vi "Export.vi"(8 "error in (no error)":errorcluster, 11 "Test Report.Template in":refnum<class "Test Report.Template.lvclass">) -> (0 "error out":errorcluster, 3 "Test Report.Template out":refnum<class "Test Report.Template.lvclass">)   [LabVIEW 2020, in "Caraya.lvlib" / "Test Report.Template.lvclass"]
uses:
  Test Report.Template.lvclass
  C:/projects/caraya/src/classes/Test Report/Test Report.lvclass
  Test Report.Template.lvclass/Test Report.Template.ctl
  Test Report/Test Report.lvclass
  Test Result/Test Result.lvclass
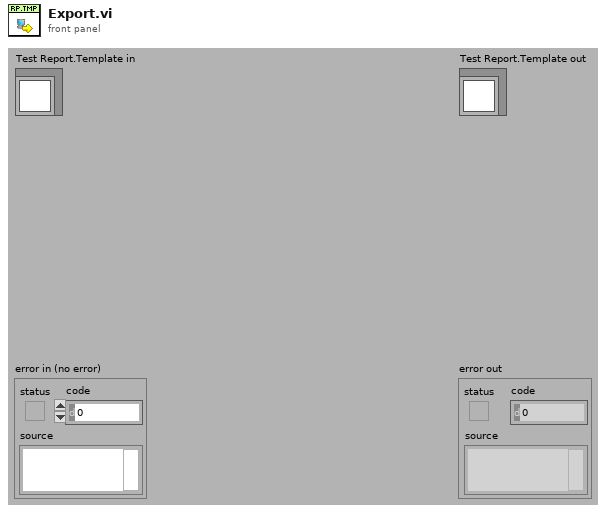
[diagram p1: front panel]
types:
  T1 = enum16{"open", "replace", "create", "open or create", "replace or create", "replace or create with confirmation"}
  T2 = typedef "Caraya.lvlib/Test Result.lvclass/Assert Event Data (Extended).ctl" = cluster{"name":string, "passed":bool, "call-chain":string[], "test-error":errorcluster, "timestamp":timestamp, "assert-id":string, "test-id":string, "time":dbl, "message":string, "properties":variant, "measurements":variant, "user-defined":variant}
  T3 = typedef "Caraya.lvlib/Test Result.lvclass/Test Node (Extended).ctl" = cluster{"Test Registration":T4, "Defined":bool, "Passed":bool, "properties":variant}
  T4 = typedef "Caraya.lvlib/Test Result.lvclass/Test Registration Data.ctl" = cluster{"Name":string, "Call Chain":string[], "Time Stamp":timestamp, "Test ID":string, "Caller ID":string}
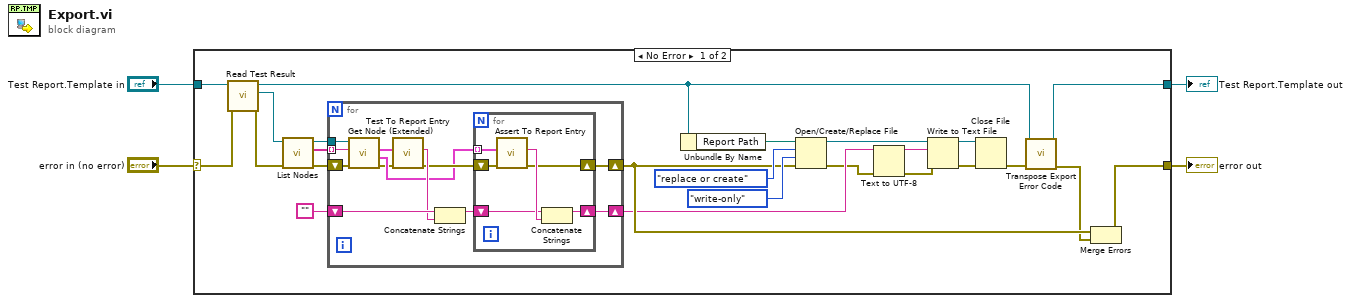
[diagram p0: block diagram]
diagram:
  n1 = case shown="No Error" "error in (no error)" {
    selector: "error in (no error)" -> [w21 w48]
    tunnel: [w13 w48] -> w3
    tunnel: [w10 w47] -> w1
    tunnel: "Test Report.Template in" -> [w22 w47]
    frame No Error {
      n2 = call "Read Test Result.vi"("error in (no error)"=w21, "Test Report in"=w22) -> ("error out"=w15:errorcluster, "Caraya.lvlib:Test Result.lvclass"=w20:refnum<class "Test Result.lvclass">, "Test Report out"=w11:refnum<class "Test Report.Template.lvclass">)  [unwired: 7 in]
      n3 = call "List Nodes.vi"("error in (no error)"=w15, "Test Result in"=w20) -> ("error out"=w16:errorcluster, "Nodes"=w19:string[], "Test Result out"=w18:refnum<class "Test Result.lvclass">)  [unwired: 7 in]
      n4 = for {
        tunnel: w19 -> [w33] mode=indexing
        tunnel: w18 -> [w34]
        shift-right: [w37] -> w8
        shift-left: "" -> [w40]
        shift-right: [w35] -> w14
        shift-left: w16 -> [w30]
        n5 = call "Get Node (Extended).vi"("error in (no error)"=w30, "Node"=w33, "Test Result in"=w34) -> ("error out"=w29:errorcluster, "Assertions"=w31:T2[], "Test Node"=w32:T3)  [unwired: 3 in, 3 out]
        n6 = call "Test To Report Entry.vi"("error in (no error)"=w29, "Test Node"=w32) -> ("error out"=w36:errorcluster, "String"=w39:string)  [unwired: 8 in]
        n7 = Concatenate Strings(w40, w39) -> (w38:string)
        n8 = for {
          shift-right: [w43] -> w37
          shift-left: w38 -> [w44]
          tunnel: w31 -> [w46] mode=indexing
          shift-right: [w41] -> w35
          shift-left: w36 -> [w42]
          n9 = call "Assert To Report Entry.vi"("error in (no error)"=w42, "Assert Event Data"=w46) -> ("error out"=w41:errorcluster, "String"=w45:string)  [unwired: 8 in]
          n10 = Concatenate Strings(w44, w45) -> (w43:string)
        }
      }
      n11 = Unbundle By Name(w11) -> ("Report Path"=w23:path)
      n12 = Open/Create/Replace File(file path (use dialog)=w23, error in=w14, operation (0:open)=T1."replace or create", access (0:read/write)=enum16{"read/write", "read-only", "write-only"}."write-only") -> (refnum out=w26:refnum<file>, error out=w6:errorcluster)  [unwired: 2 in, 1 out]
      n13 = Text to UTF-8(8:w6, 11:w8) -> (0:w5:errorcluster, 3:w7:string)  [unwired: 1 in]
      n14 = Write to Text File(file (use dialog)=w26, text=w7, error in=w5) -> (refnum out=w25:refnum<file>, error out=w24:errorcluster)  [unwired: 1 in, 1 out]
      n15 = Close File(refnum=w25, error in=w24) -> (error out=w12:errorcluster)  [unwired: 1 out]
      n16 = call-dynamic "Transpose Export Error Code.vi"("error in (no error)"=w12, "Test Report"=w11) -> ("error out"=w9:errorcluster, "Test Report out"=w10:refnum<class "Test Report.Template.lvclass">)  [unwired: 8 in]
      n17 = Merge Errors(w14, w9) -> (w13:errorcluster)
    }
    frame Error {
    }
  }
  "error out" <- w3
  "Test Report.Template out" <- w1
